vi "ZM-CP-MX-initAll.vi"(8 "error in (no error)":errorcluster, 11 "ZM-CP-communication_protocol in":refnum<class "ZM-CP-communication_protocol.lvclass">) -> (0 "error out":errorcluster, 3 "ZM-CP-communication_protocol out":refnum<class "ZM-CP-communication_protocol.lvclass">)   [LabVIEW 2020, in "ZM-CP-MX-multi_protocol.lvlib" / "ZM-CP-MX-multi_protocol.lvclass"]
doc: "Hook of the multi protocol, called by its ZM-CP-init override after Call Parent: initialises every protocol in the array in order and stops at the first error, which is returned. The array keeps its length. Reentrant, because an element can itself be a multi protocol."
uses:
  ZM-CP-MX-multi_protocol.lvclass
  ZM-CP-communication_protocol/ZM-CP-communication_protocol/ZM-CP-communication_protocol.lvclass
  ZM-CP-MX-multi_protocol.lvclass/ZM-CP-MX-multi_protocol.ctl
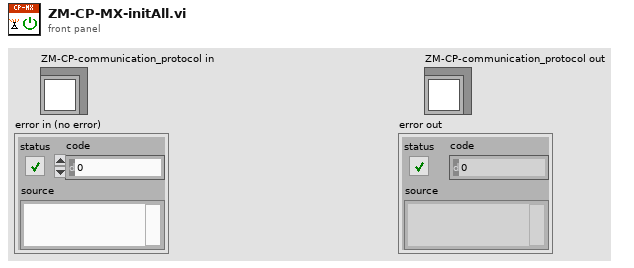
[diagram p1: front panel]
types:
  T1 = typedef "ZM-CP-MX-multi_protocol.lvlib/ZM-CP-MX-multi_protocol.lvclass/ZM-CP-MX-PROTOCOLS.ctl" = refnum<class "ZM-CP-communication_protocol.lvclass">[]
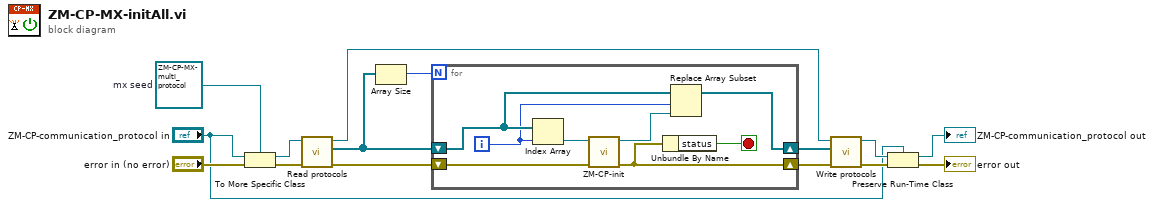
[diagram p0: block diagram]
diagram:
  w14 = refnum<class "ZM-CP-MX-multi_protocol.lvclass"> refnum  # mx seed
  n1 = To More Specific Class(target class=w14, reference="ZM-CP-communication_protocol in", error in="error in (no error)") -> (specific class reference=w12:refnum<class "ZM-CP-MX-multi_protocol.lvclass">, error out=w13:errorcluster)
  n2 = call "Read protocols.vi"("error in (no error)"=w13, "ZM-CP-MX-multi_protocol in"=w12) -> ("error out"=w10:errorcluster, "ZM-CP-MX-PROTOCOLS"=w11:T1, "ZM-CP-MX-multi_protocol out"=w8:refnum<class "ZM-CP-MX-multi_protocol.lvclass">)  [unwired: 7 in]
  n3 = Array Size(array=w11) -> (size(s)=w9:i32)
  n4 = for {
    N: w9 -> [_]
    shift-right: [w19] -> w7
    shift-left: w11 -> [w21]
    shift-right: [w18] -> w6
    shift-left: w10 -> [w22]
    i -> [w16]
    stop <- w17 stop-if-true
    n5 = Index Array(array=w21, index=w16) -> (element=w23:refnum<class "ZM-CP-communication_protocol.lvclass">)
    n6 = call-dynamic "ZM-CP-init.vi"("error in (no error)"=w22, "ZM-CP-communication_protocol in"=w23) -> ("error out"=w18:errorcluster, "ZM-CP-communication_protocol out"=w20:refnum<class "ZM-CP-communication_protocol.lvclass">)  [unwired: 8 in]
    n7 = Unbundle By Name(w18) -> ("status"=w17:bool)
    n8 = Replace Array Subset(array=w21, new element=w20, index=w16) -> (w19:T1)
  }
  n9 = call "Write protocols.vi"("error in (no error)"=w6, "ZM-CP-MX-PROTOCOLS"=w7, "ZM-CP-MX-multi_protocol in"=w8) -> ("error out"=w4:errorcluster, "ZM-CP-MX-multi_protocol out"=w5:refnum<class "ZM-CP-MX-multi_protocol.lvclass">)  [unwired: 7 in]
  n10 = Preserve Run-Time Class(object in=w5, error in=w4, 2:"ZM-CP-communication_protocol in") -> (object out=→"ZM-CP-communication_protocol out":refnum<class "ZM-CP-communication_protocol.lvclass">, error out=→"error out":errorcluster)
